vi "enqueue_dequeue.vi"() -> ()   [LabVIEW 2016]
panel:
  out "Dequeue Chart":i32(graph)
  out "Enqueue Chart":i32(graph)
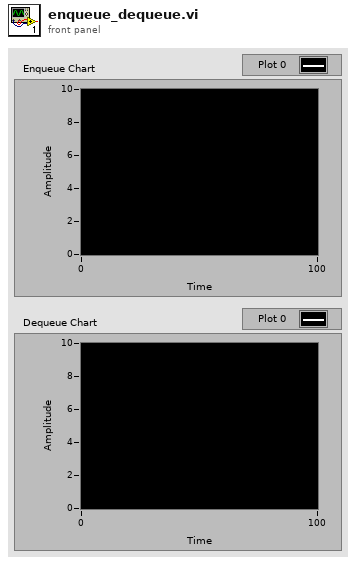
[diagram p1: front panel]
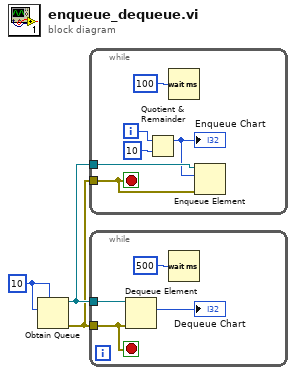
[diagram p0: block diagram]
diagram:
  w3 = 10 ("max queue size (-1, unlimited)")
  n1 = Obtain Queue(max queue size (-1, unlimited)=w3, element data type=w3) -> (queue out=w2:refnum<queue>, error out=w1:errorcluster)  [unwired: 3 in, 1 out]
  n2 = while {
    tunnel: w2 -> [w9]
    tunnel: w1 -> [w8]
    i -> [w7]
    stop <- w8 stop-if-true
    n3 = Quotient & Remainder(x=w7, y=10) -> (x-y*floor(x/y)=w5:i32)  [unwired: 1 out]
    "Enqueue Chart" <- w5
    n4 = Wait (ms)(milliseconds to wait=u32 100) -> ()  [unwired: 1 out]
    n5 = Enqueue Element(queue=w9, element=w5, error in (no error)=w8) -> ()  [unwired: 1 in, 3 out]
  }
  n6 = while {
    tunnel: w2 -> [w13]
    tunnel: w1 -> [w12]
    stop <- w12 stop-if-true
    n7 = Dequeue Element(queue=w13, error in (no error)=w12) -> (element=→"Dequeue Chart":i32)  [unwired: 1 in, 3 out]
    n8 = Wait (ms)(milliseconds to wait=u32 500) -> ()  [unwired: 1 out]
  }
